vi "Write Fetch Interval.vi"(8 "error in (no error)":errorcluster, 10 "Fetch Interval":i32, 11 "AUDIX EM1000 in":refnum<class "AUDIX EM1000.lvclass">) -> (0 "error out":errorcluster, 3 "AUDIX EM1000 out":refnum<class "AUDIX EM1000.lvclass">)   [LabVIEW 2023, in "Turn Table and Mast.lvlib" / "AUDIX EM1000.lvclass"]
uses:
  AUDIX EM1000.lvclass
  AUDIX EM1000.lvclass/AUDIX EM1000.ctl
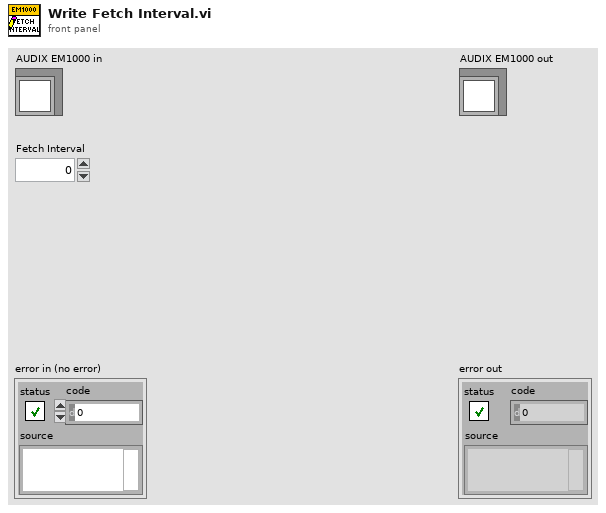
[diagram p1: front panel]
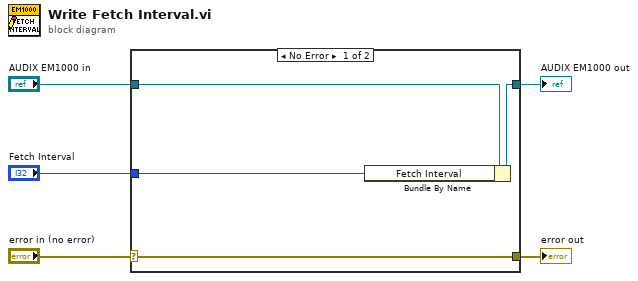
[diagram p0: block diagram]
diagram:
  n1 = case shown="No Error" "error in (no error)" {
    selector: "error in (no error)" -> [w9 w10]
    tunnel: [w9 w10] -> w4
    tunnel: [w7 w11] -> w2
    tunnel: "AUDIX EM1000 in" -> [w8 w11]
    tunnel: "Fetch Interval" -> [w6 _]
    frame No Error {
      n2 = Bundle By Name(cluster=w8, "Fetch Interval"=w6) -> (w7:refnum<class "AUDIX EM1000.lvclass">)
    }
    frame Error {
    }
  }
  "error out" <- w4
  "AUDIX EM1000 out" <- w2
